vi "Apply Event.vi"(7 "scale":dbl=1.0, 8 "other":i32, 9 "stock":i32, 10 "event":T3, 11 "market":T1) -> (3 "market out":T1)   [LabVIEW 2020, in "Full Featured MCP Server.lvlib"]
doc: "Lets one event hit the market and publishes it as news. Every stock in the scope of the event (the stock, the stock and the other one, the whole sector of the stock, or all stocks) gets the jump as a shock for the next price step and the follow as momentum that fades over the next minutes, and turns more nervous. scale multiplies jump and follow. Prices are not changed here: Move Prices applies the shock."
uses:
  Full Featured MCP Server.lvlib
  Market State.ctl
  News Item.ctl
  Event Template.ctl
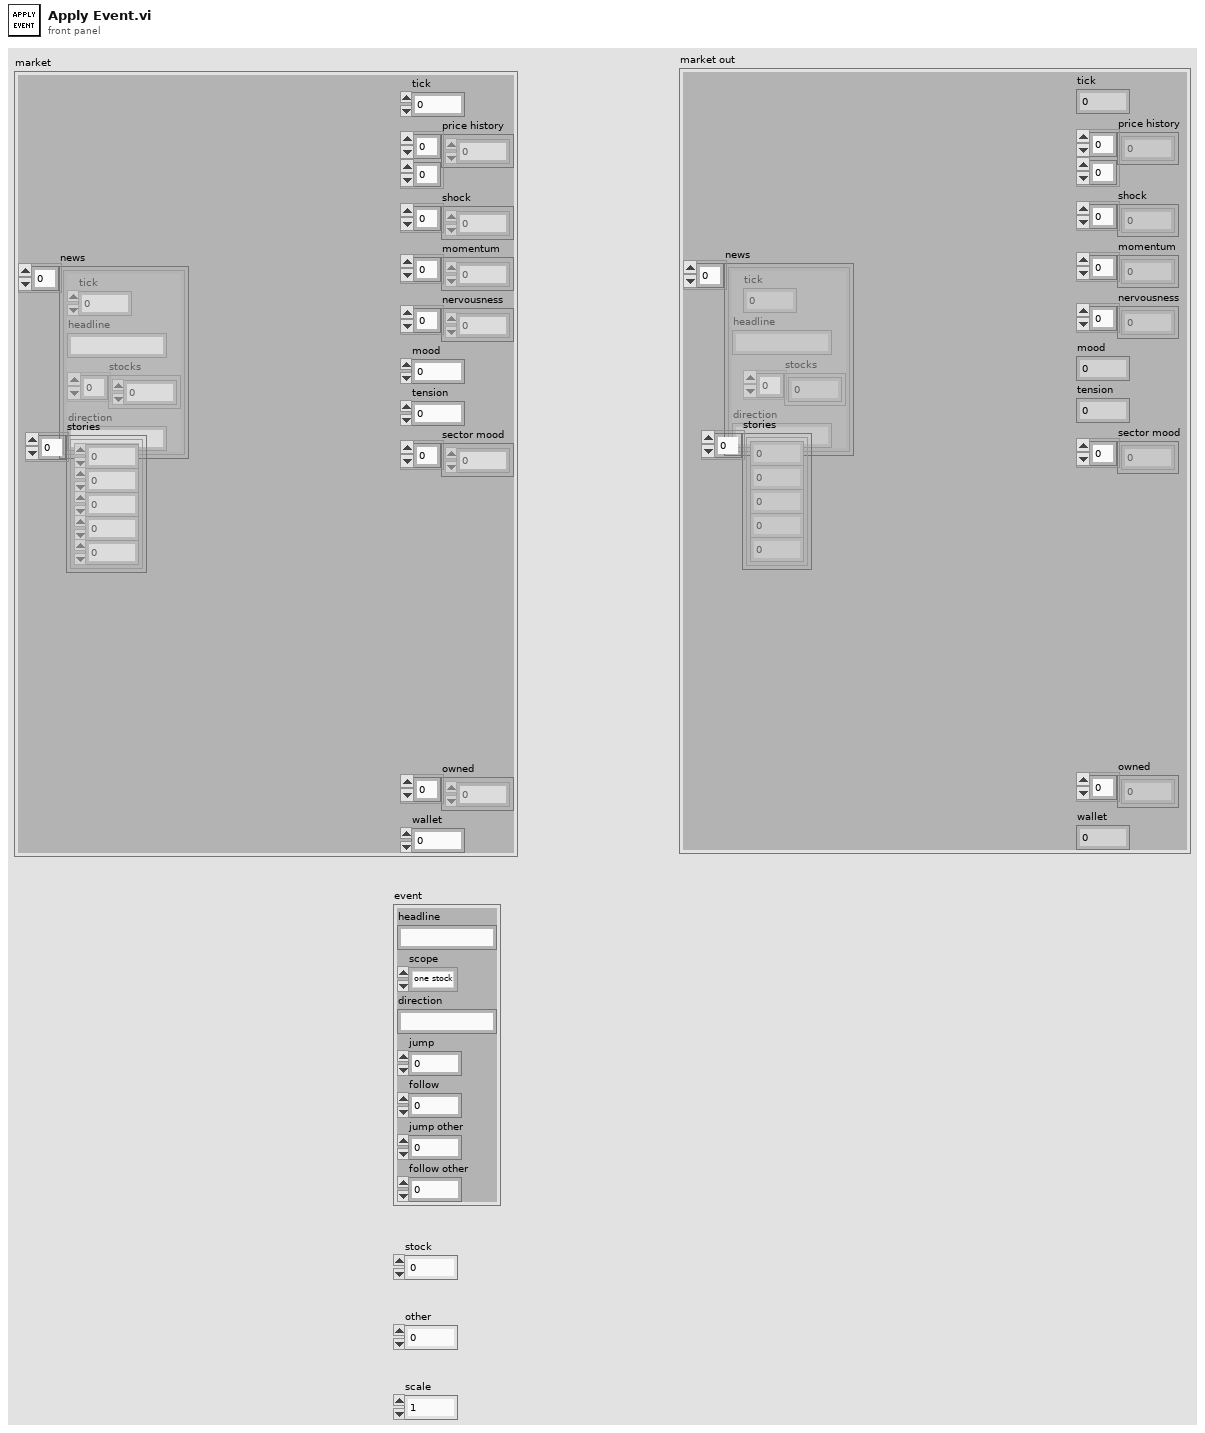
[diagram p1: front panel]
types:
  T1 = typedef "Full Featured MCP Server.lvlib/Market State.ctl" = cluster{"tick":i32, "price history":dbl[][], "shock":dbl[], "momentum":dbl[], "nervousness":dbl[], "mood":dbl, "tension":dbl, "sector mood":dbl[], "news":T2[], "stories":cluster{"arc":i32, "step":i32, "due":i32, "stock":i32, "other":i32}[], "owned":i32[], "wallet":dbl}
  T2 = typedef "Full Featured MCP Server.lvlib/News Item.ctl" = cluster{"tick":i32, "headline":string, "stocks":i32[], "direction":string}
  T3 = typedef "Full Featured MCP Server.lvlib/Event Template.ctl" = cluster{"headline":string, "scope":enum16{"one stock", "two stocks", "sector", "market"}, "direction":string, "jump":dbl, "follow":dbl, "jump other":dbl, "follow other":dbl}
  T4 = enum16{"one stock", "two stocks", "sector", "market"}
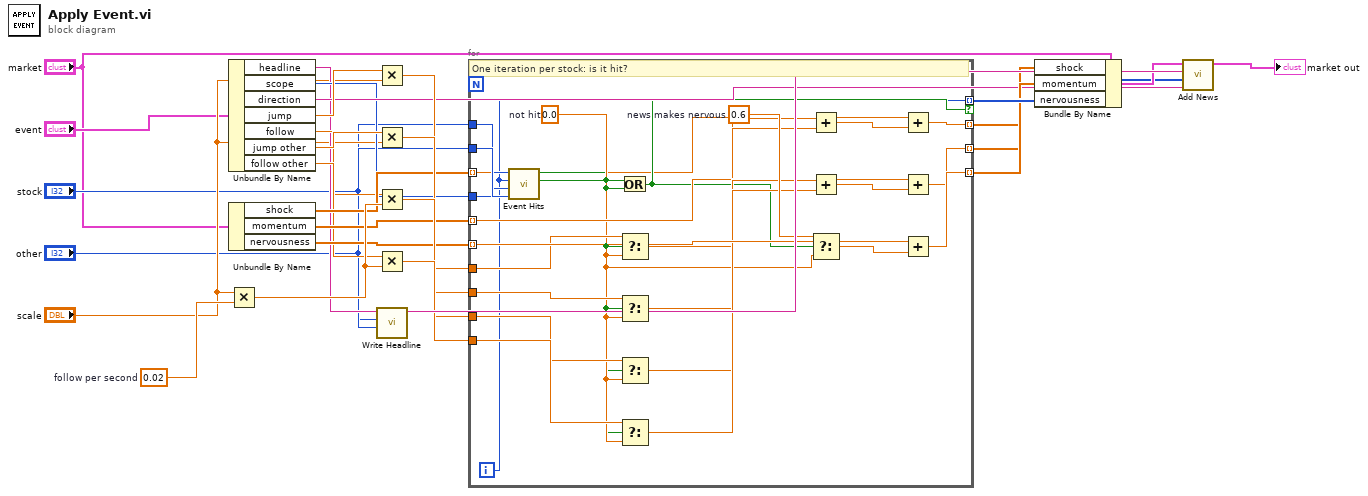
[diagram p0: block diagram]
diagram:
  w16 = 0.02  # follow per second
  n1 = Unbundle By Name("event") -> ("headline"=w6:string, "scope"=w7:T4, "direction"=w8:string, "jump"=w9:dbl, "follow"=w10:dbl, "jump other"=w11:dbl, "follow other"=w12:dbl)
  n2 = Unbundle By Name("market") -> ("shock"=w13:dbl[], "momentum"=w14:dbl[], "nervousness"=w15:dbl[])
  n3 = Multiply(x="scale", y=w16) -> (x*y=w17:dbl)
  n4 = Multiply(x=w9, y="scale") -> (x*y=w18:dbl)
  n5 = Multiply(x=w11, y="scale") -> (x*y=w19:dbl)
  n6 = Multiply(x=w10, y=w17) -> (x*y=w20:dbl)
  n7 = Multiply(x=w12, y=w17) -> (x*y=w21:dbl)
  n8 = call "Write Headline.vi"("other"="other", "stock"="stock", "template"=w6) -> ("headline"=w27:string)  [unwired: 8 in]
  n9 = for {
    tunnel: "stock" -> [w32]
    tunnel: "other" -> [w33]
    tunnel: [w29] -> w25 mode=indexing if=w37
    tunnel: w13 -> [w30] mode=indexing
    tunnel: w7 -> [w31]
    tunnel: w14 -> [w44] mode=indexing
    tunnel: w15 -> [w51] mode=indexing
    tunnel: w18 -> [w38]
    tunnel: w19 -> [w40]
    tunnel: w20 -> [w45]
    tunnel: w21 -> [w47]
    tunnel: [w43] -> w22 mode=indexing
    tunnel: [w50] -> w23 mode=indexing
    tunnel: [w54] -> w24 mode=indexing
    i -> [w29]
    w52 = 0.6  # news makes nervous
    w36 = 0.0  # not hit
    # "One iteration per stock: is it hit?"
    n10 = call "Event Hits.vi"("other"=w33, "stock"=w32, "candidate"=w29, "scope"=w31) -> ("as other?"=w35:bool, "as stock?"=w34:bool)  [unwired: 6 in]
    n11 = Or(x=w34, y=w35) -> (x .or. y?=w37:bool)
    n12 = Select(t=w38, s=w34, f=w36) -> (s? t:f=w39:dbl)
    n13 = Select(t=w40, s=w35, f=w36) -> (s? t:f=w41:dbl)
    n14 = Select(t=w45, s=w34, f=w36) -> (s? t:f=w46:dbl)
    n15 = Select(t=w47, s=w35, f=w36) -> (s? t:f=w48:dbl)
    n16 = Add(x=w39, y=w41) -> (x+y=w42:dbl)
    n17 = Add(x=w46, y=w48) -> (x+y=w49:dbl)
    n18 = Select(t=w52, s=w37, f=w36) -> (s? t:f=w53:dbl)
    n19 = Add(x=w30, y=w42) -> (x+y=w43:dbl)
    n20 = Add(x=w44, y=w49) -> (x+y=w50:dbl)
    n21 = Add(x=w51, y=w53) -> (x+y=w54:dbl)
  }
  n22 = Bundle By Name(cluster="market", "shock"=w22, "momentum"=w23, "nervousness"=w24) -> (w26:T1)
  n23 = call "Add News.vi"("direction"=w8, "stocks"=w25, "headline"=w27, "market"=w26) -> ("market out"=→"market out":T1)  [unwired: 7 in]
